vi "Start VI Helpeks.vi"() -> ()   [LabVIEW 2014]
doc: "::: VI Helpeks :::\nCopyright (c) 2000-2026 Konstantin Shifershteyn. All rights reserved."
uses:
  <vilib>/Utility/sysdir.llb/System Directory Type.ctl
  <vilib>/Platform/browser.llb/Open URL in Default Browser (string).vi
panel:
  out "LV Version":string="."
  out "Progress":i32(slide)=-1 caption="Loading . . ." scale=-1.0..380.0
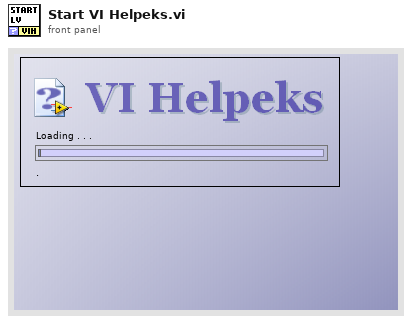
[diagram p1: front panel]
types:
  T1 = cluster{"Left Button Key Shortcut":cluster{"Control":bool, "Shift":bool, "Key":string}, "Center Button Key Shortcut":cluster{"Control":bool, "Shift":bool, "Key":string}, "Right Button Key Shortcut":cluster{"Control":bool, "Shift":bool, "Key":string}}
  T2 = enum32{"Invalid", "Standard", "Closed", "Hidden", "Minimized", "Maximized"}
  T3 = typedef "System Directory Type.ctl" = i32
  T4 = enum16{"Left Button", "Center Button", "Right Button", "Window Close"}
  T5 = typedef "NI_FileType.lvlib/LVFileType.ctl" = enum32{"Invalid file", "Unknown type", "Instrument", "Control", "Polymorphic VI", "Project", "Library", "LVClass", "XControl", "XNode", "Shared library", ".NET assembly", "ActiveX interface", "CIN", "Run-time menu", "Palette menu", "Help file", "LLB", "XNode Edit Dependency", "Class Private Data Control", "Statechart", "MathScript .m file", "Ladder Diagram", "LVLibp", "XNode Build Dependency"}
  T6 = cluster{"path":path, "delimited name":string, "type":T5, "iState":u32, "iStyle":u16, "wStyle":u16, "buttons":u16, "viflags":u32, "viflags2":u32, "links":u32[]}[]
  T7 = enum32{"Bad", "Idle", "Run top level", "Running"}
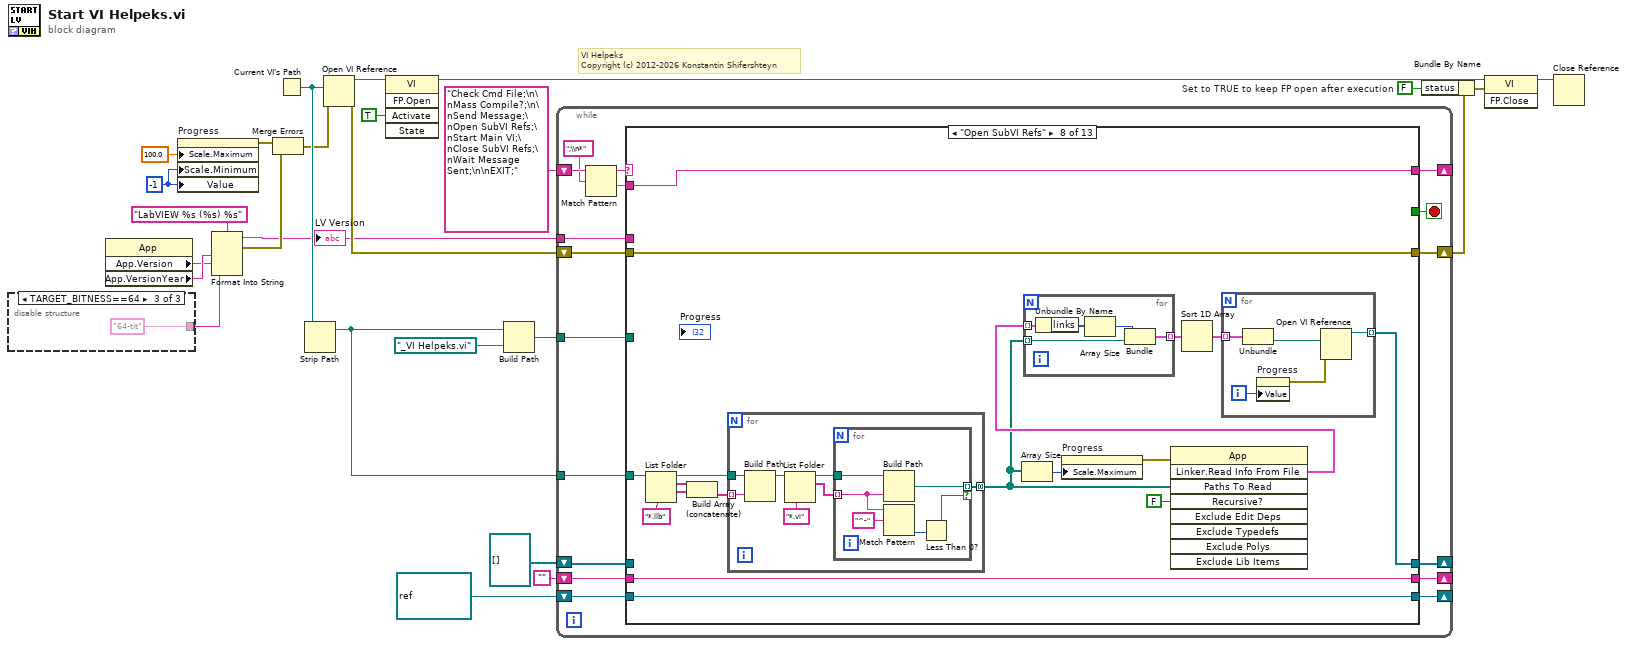
[diagram p0: block diagram]
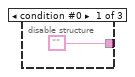
[diagram p2: hidden frame]
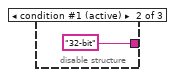
[diagram p3: hidden frame]
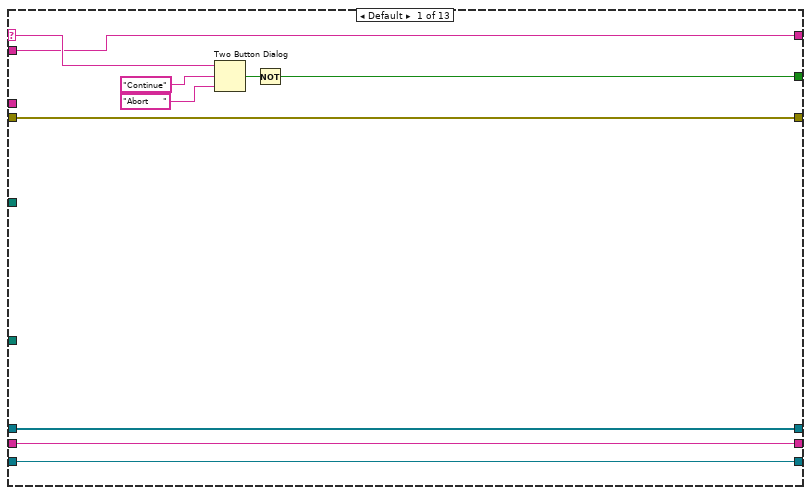
[diagram p4: hidden frame]
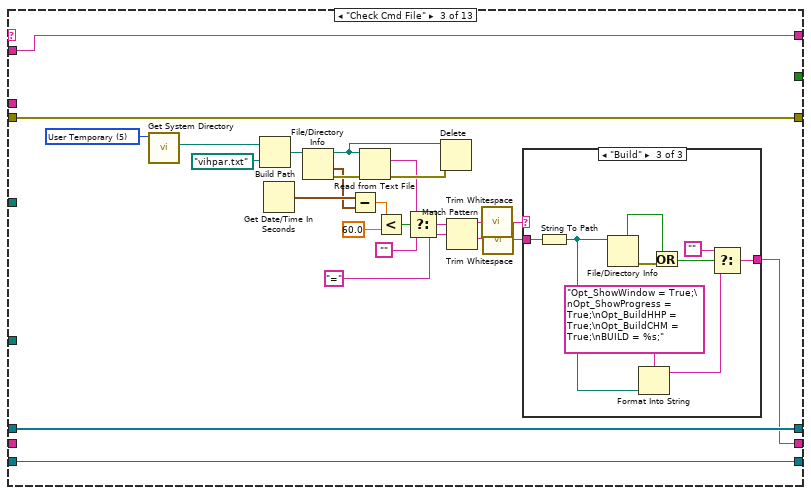
[diagram p6: hidden frame]
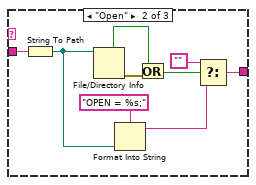
[diagram p8: hidden frame]
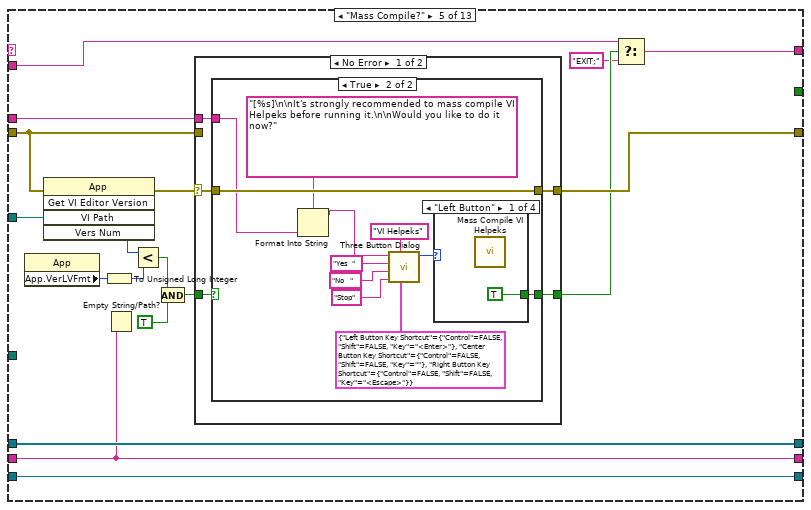
[diagram p10: hidden frame]
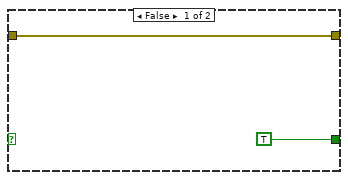
[diagram p11: hidden frame]
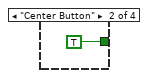
[diagram p12: hidden frame]
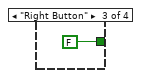
[diagram p13: hidden frame]
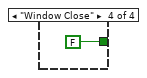
[diagram p14: hidden frame]
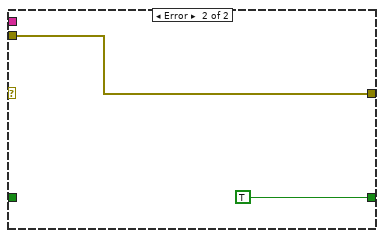
[diagram p15: hidden frame]
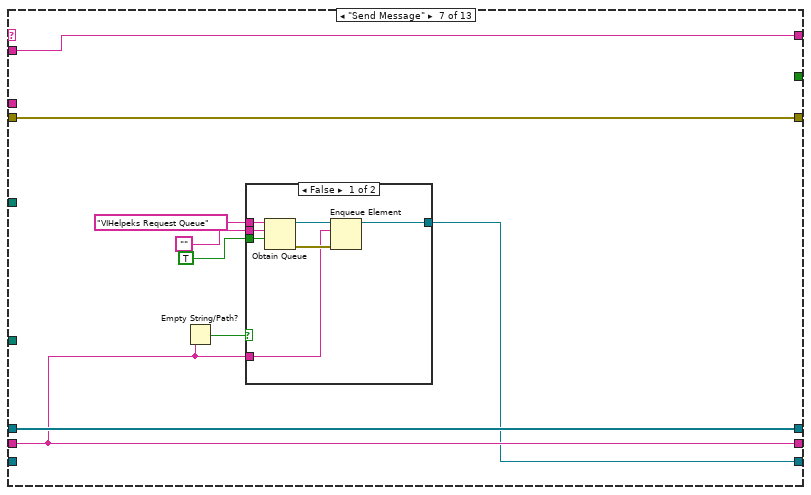
[diagram p17: hidden frame]
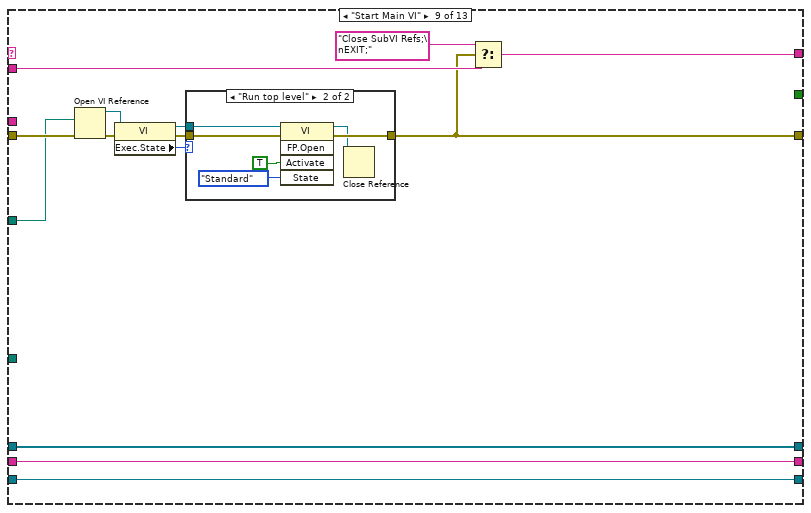
[diagram p19: hidden frame]
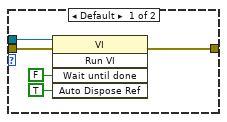
[diagram p20: hidden frame]
diagram:
  w18 = -1 ("Progress")
  w23 = FALSE  # Set to TRUE to keep FP open after execution
  # "VI Helpeks\nCopyright (c) 2012-2026 Konstantin Shifershteyn"
  n1 = disable-structure shown="TARGET_BITNESS==64" {
    disable-tunnel: ["" "32-bit" "64-tit"] -> w6
    frame condition #0 {
    }
    frame condition #1 (active) {
    }
    frame condition #2 {
    }
  }
  n2 = property class="App"() -> ("App.Version"=w9:string, "App.VersionYear"=w10:string)  [unwired: 2 in, 2 out]
  n3 = property on="Progress" class="Slide (strict)"("Scale.Maximum"=100.0 ("Scale.Range:Maximum"), "Scale.Minimum"=w18, "Value"=w18) -> (error out=w17:errorcluster)  [unwired: 2 in, 1 out]
  n4 = Format Into String(format string="LabVIEW %s (%s) %s" ("string"), w10, w9, w6) -> (resulting string=w2:string, error out=w12:errorcluster)  [unwired: 2 in]
  "LV Version" <- w2
  n5 = Merge Errors(w17, w12) -> (w13:errorcluster)
  n6 = Current VI's Path() -> (path=w26:path)
  n7 = Strip Path(path=w26) -> (stripped path=w1:path)  [unwired: 1 out]
  n8 = Open VI Reference(vi path=w26, error in (no error)=w13) -> (vi reference=w5:refnum<vi>, error out=w20:errorcluster)  [unwired: 4 in]
  n9 = invoke class="VI" method="FP.Open"(reference=w5, "Activate"=TRUE ("Activate?")) -> (reference out=w4:refnum<vi>)  [unwired: 3 in, 4 out]
  n10 = Build Path(base path=w1, name or relative path=path "_VI Helpeks.vi") -> (appended path=w21:path)
  n11 = while {
    tunnel: w21 -> [w44]
    tunnel: w1 -> [w43]
    shift-right: [w46] -> w25
    shift-left: w20 -> [w45]
    shift-right: [w42] -> _
    shift-left: refnum<vi>[] [] -> [w41]
    shift-right: [w38] -> _
    shift-left: "Check Cmd File;\n\nMass Compile?;\n\nSend Message;\nOpen SubVI Refs;\nStart Main VI;\nClose SubVI Refs;\nWait Message Sent;\n\nEXIT;" -> [w40]
    shift-right: [w33] -> _
    shift-left: "" -> [w34]
    shift-right: [w32] -> _
    shift-left: refnum<queue> refnum ("queue out") -> [w31]
    tunnel: w2 -> [w30]
    stop <- w35 stop-if-true
    n12 = Match Pattern(string=w40, regular expression=";\\n*") -> (before substring=w39:string, after substring=w37:string)  [unwired: 1 in, 2 out]
    n13 = case shown="\"Open SubVI Refs\"" w39 {
      selector: w39 -> [w55 _ _ _ _ _ _ _ _ _ _ _ _]
      tunnel: [w56 w60 w86 w108 w121 w155 w163 w184 w217 w242 w249 w276 w278] -> w46
      tunnel: w45 -> [w56 w60 w86 w108 w122 w155 w163 w184 w227 w242 w249 w276 w278]
      tunnel: w44 -> [_ _ _ _ w116 _ _ _ w226 _ _ _ _]
      tunnel: w43 -> [_ _ _ _ _ _ _ w177 _ _ _ _ _]
      tunnel: [w54 w59 w84 w107 w127 w154 w165 w185 w220 refnum<vi>[] [] w251 w275 w283] -> w42
      tunnel: w41 -> [w54 w59 w84 w107 w127 w154 w165 _ w220 w244 w251 w275 w283]
      tunnel: [w53 w61 w85 w109 w118 w156 w164 w181 w218 w241 w250 w277 w281] -> w38
      tunnel: w37 -> [w53 w61 w85 w109 w119 w156 w164 w181 w219 w241 w250 w277 w281]
      tunnel: [w49 _ _ _ _ _ _ _ _ _ _ _ TRUE] -> w35
      tunnel: w34 -> [w51 w58 _ w106 w113 w153 w162 w180 w215 w240 w247 w274 w280]
      tunnel: [w51 w58 w65 w106 w113 w153 w162 w180 w215 w240 w247 w274 w280] -> w33
      tunnel: [w47 w57 w64 w105 w111 w152 w157 w179 w214 w239 w246 w273 w279] -> w32
      tunnel: w31 -> [w47 w57 w64 w105 w111 w152 _ w179 w214 w239 w246 w273 w279]
      tunnel: w30 -> [_ _ _ _ w110 _ _ _ _ _ _ _ _]
      frame Default {
        n14 = Two Button Dialog(message=w55, 1:"Abort     ", 2:"Continue") -> (T button?=w52:bool)
        n15 = Not(x=w52) -> (.not. x?=w49:bool)
      }
      frame "" {
      }
      frame "Check Cmd File" {
        w62 = T3 5 items=["User Home"=0, "User Desktop"=1, "User Documents"=2, "User Application Data"=3, "User Preferences"=4, "User Temporary"=5, "Public Documents"=6, "Public Application Data"=7, "Public Preferences"=8, "Public Cache"=13, "System Core Libraries"=9, "System Installed Libraries"=10, "Application Files"=11, "Boot Volume Root"=12] ("system directory type")
        n16 = call <vilib>:"Get System Directory.vi"("system directory type"=w62) -> ("system directory"=w63:path)  [unwired: 10 in]
        n17 = Build Path(base path=w63, name or relative path=path "vihpar.txt") -> (appended path=w82:path)
        n18 = Get Date/Time In Seconds() -> (seconds since 1Jan1904=w78:timestamp)
        n19 = File/Directory Info(path=w82) -> (path out=w80:path, last mod=w77:timestamp, error out=w81:errorcluster)  [unwired: 1 in, 4 out]
        n20 = Subtract(x=w78, y=w77) -> (x-y=w76:dbl)
        n21 = Read from Text File(file (use dialog)=w80, error in=w81) -> (text=w73:string, error out=w79:errorcluster)  [unwired: 2 in, 2 out]
        n22 = Less?(x=w76, y=60.0) -> (x < y?=w74:bool)
        n23 = Select(t=w73, s=w74, f="") -> (s? t:f=w71:string)
        n24 = Delete(path (use dialog)=w80, error in=w79) -> ()  [unwired: 3 in, 3 out]
        n25 = Match Pattern(string=w71, regular expression="=") -> (before substring=w69:string, after substring=w67:string)  [unwired: 1 in, 2 out]
        n26 = call <vilib>:"Trim Whitespace.vi"("string"=w69) -> ("trimmed string"=w68:string)  [unwired: 1 in]
        n27 = call <vilib>:"Trim Whitespace.vi"("string"=w67) -> ("trimmed string"=w66:string)  [unwired: 1 in]
        n28 = case shown="\"Build\"" w68 {
          tunnel: w66 -> [_ w95 w104]
          tunnel: [_ w91 w100] -> w65
          frame Default {
          }
          frame "Open" {
            n29 = String To Path(string=w95) -> (path=w90:path)
            n30 = File/Directory Info(path=w90) -> (directory=w87:bool, error out=w89:errorcluster)  [unwired: 1 in, 5 out]
            n31 = Format Into String(format string="OPEN = %s;", w90) -> (resulting string=w93:string)  [unwired: 2 in, 1 out]
            n32 = Or(x=w87, y=w89) -> (x .or. y?=w88:bool)
            n33 = Select(t="", s=w88, f=w93) -> (s? t:f=w91:string)
          }
          frame "Build" {
            n34 = String To Path(string=w104) -> (path=w99:path)
            n35 = File/Directory Info(path=w99) -> (directory=w96:bool, error out=w98:errorcluster)  [unwired: 1 in, 5 out]
            n36 = Format Into String(format string="Opt_ShowWindow = True;\nOpt_ShowProgress = True;\nOpt_BuildHHP = True;\nOpt_BuildCHM = True;\nBUILD = %s;", w99) -> (resulting string=w102:string)  [unwired: 2 in, 1 out]
            n37 = Or(x=w96, y=w98) -> (x .or. y?=w97:bool)
            n38 = Select(t="", s=w97, f=w102) -> (s? t:f=w100:string)
          }
        }
      }
      frame "--------------------- 1" {
      }
      frame "Mass Compile?" {
        n39 = property class="App"() -> ("App.VerLVFmt"=w125:i32)  [unwired: 2 in, 2 out]
        n40 = invoke class="App" method="Get VI Editor Version"(error in=w122, "VI Path"=w116) -> (error out=w123:errorcluster, "Vers Num"=w124:u32)  [unwired: 3 in, 3 out]
        n41 = To Unsigned Long Integer(number=w125) -> (unsigned 32bit integer=w126:u32)
        n42 = Empty String/Path?(string/path=w113) -> ()  [unwired: 1 out]
        n43 = Less?(x=w124, y=w126) -> (x < y?=w115:bool)
        n44 = And(x=w115, y=TRUE) -> (x .and. y?=w114:bool)
        n45 = case shown="No Error" w123 {
          selector: w123 -> [w130 _]
          tunnel: w114 -> [w132 _]
          tunnel: [w131 w151] -> w121
          tunnel: w122 -> [_ w151]
          tunnel: [w129 TRUE] -> w120
          tunnel: w110 -> [w128 _]
          frame No Error {
            n46 = case shown="True" w132 {
              tunnel: [w134 w145] -> w131
              tunnel: w130 -> [w134 w145]
              tunnel: [TRUE w139] -> w129
              tunnel: w128 -> [_ w135]
              frame False {
              }
              frame True {
                n47 = Format Into String(format string="[%s]\n\nIt's strongly recommended to mass compile VI Helpeks before running it.\n\nWould you like to do it now?", w135) -> (resulting string=w137:string)  [unwired: 2 in, 1 out]
                n48 = call <vilib>:"Three Button Dialog.vi"("Keyboard Shortcuts (Left is <Enter>)"=T1 {"Left Button Key Shortcut"={"Control"=FALSE, "Shift"=FALSE, "Key"="<Enter>"}, "Center Button Key Shortcut"={"Control"=FALSE, "Shift"=FALSE, "Key"=""}, "Right Button Key Shortcut"={"Control"=FALSE, "Shift"=FALSE, "Key"="<Escape>"}}, "Window Title (\"\")"="VI Helpeks" ("Window Title (\"\")"), "Right Button Text (\"Cancel\")"="Stop" ("Right Button Text (\"Cancel\")"), "Center Button Text (\"No\")"="No   " ("F button name (\"Cancel\")"), "Left Button Text (\"Yes\")"="Yes  " ("T button name (\"OK\")"), "message"=w137) -> ("Which Button?"=w144:T4)  [unwired: 5 in]
                n49 = case shown="\"Left Button\"" w144 {
                  tunnel: [TRUE TRUE FALSE FALSE] -> w139
                  frame "Left Button" {
                    n50 = call "Mass Compile VI Helpeks.vi"() -> ()  [unwired: 1 in]
                  }
                  frame "Center Button" {
                  }
                  frame "Right Button" {
                  }
                  frame "Window Close" {
                  }
                }
              }
            }
          }
          frame Error {
          }
        }
        n51 = Select(t=w119, s=w120, f="EXIT;") -> (s? t:f=w118:string)
      }
      frame "--------------------- 2" {
      }
      frame "Send Message" {
        n52 = Empty String/Path?(string/path=w162) -> (empty?=w158:bool)
        n53 = case shown="False" w158 {
          tunnel: "VIHelpeks Request Queue" -> [w172 _]
          tunnel: "" -> [w171 _]
          tunnel: TRUE -> [w170 _]
          tunnel: w162 -> [w167 _]
          tunnel: [w166 _] -> w157
          frame False {
            n54 = Obtain Queue(name (unnamed)=w172, element data type=w171, create if not found? (T)=w170) -> (queue out=w169:refnum<queue>, error out=w168:errorcluster)  [unwired: 2 in, 1 out]
            n55 = Enqueue Element(queue=w169, element=w167, error in (no error)=w168) -> (queue out=w166:refnum<queue>)  [unwired: 1 in, 2 out]
          }
          frame True {
          }
        }
      }
      frame "Open SubVI Refs" {
        n56 = List Folder(path=w177, pattern="*.llb") -> (path out=w176:path, filenames=w175:string[], folder names=w174:string[])  [unwired: 2 in, 1 out]
        n57 = Build Array (concatenate)(w175, w174) -> (w173:string[])
        n58 = for {
          tunnel: [w194] -> w182 mode=concatenating
          tunnel: w176 -> [w193]
          tunnel: w173 -> [w191] mode=indexing
          n59 = Build Path(base path=w193, name or relative path=w191) -> (appended path=w192:path)
          n60 = List Folder(path=w192, pattern="*.vi") -> (path out=w197:path, filenames=w195:string[])  [unwired: 2 in, 2 out]
          n61 = for {
            tunnel: w197 -> [w203]
            tunnel: w195 -> [w201] mode=indexing
            tunnel: [w202] -> w194 mode=indexing if=w198
            n62 = Build Path(base path=w203, name or relative path=w201) -> (appended path=w202:path)
            n63 = Match Pattern(string=w201, regular expression="^-") -> (offset past match=w199:i32)  [unwired: 1 in, 3 out]
            n64 = Less Than 0?(x=w199) -> (x < 0?=w198:bool)
          }
        }
        n65 = Array Size(array=w182) -> (size(s)=w190:i32)
        n66 = property on="Progress" class="Slide (strict)"("Scale.Maximum"=w190) -> (error out=w187:errorcluster)  [unwired: 2 in, 1 out]
        n67 = invoke class="App" method="Linker.Read Info From File"(error in=w187, "Paths To Read"=w182, "Recursive?"=FALSE) -> ("Linker.Read Info From File"=w183:T6)  [unwired: 6 in, 8 out]
        n68 = for {
          tunnel: w183 -> [w213] mode=indexing
          tunnel: w182 -> [w211] mode=indexing
          tunnel: [w209] -> w188 mode=indexing
          n69 = Unbundle By Name(w213) -> ("links"=w212:u32[])
          n70 = Array Size(array=w212) -> (size(s)=w210:i32)
          n71 = Bundle(w210, "appended path"=w211) -> (w209:cluster{i32, "appended path":path})  [unwired: 1 in]
        }
        n72 = Sort 1D Array(array=w188) -> (sorted array=w186:cluster{i32, "appended path":path}[])
        n73 = for {
          tunnel: w186 -> [w208] mode=indexing
          tunnel: [w204] -> w185 mode=indexing
          i -> [w206]
          n74 = Unbundle(w208) -> ("appended path"=w207:path)  [unwired: 1 out]
          n75 = property on="Progress" class="Slide (strict)"("Value"=w206) -> (error out=w205:errorcluster)  [unwired: 2 in, 1 out]
          n76 = Open VI Reference(vi path=w207, error in (no error)=w205) -> (vi reference=w204:refnum<vi>)  [unwired: 4 in, 1 out]
        }
      }
      frame "Start Main VI" {
        n77 = Open VI Reference(vi path=w226, error in (no error)=w227) -> (vi reference=w224:refnum<vi>, error out=w225:errorcluster)  [unwired: 4 in]
        n78 = property class="VI"(reference=w224, error in=w225) -> (reference out=w221:refnum<vi>, error out=w222:errorcluster, "Exec.State"=w223:T7)
        n79 = case shown="\"Run top level\"" w223 {
          tunnel: [w228 w238] -> w217
          tunnel: w222 -> [w230 w234]
          tunnel: w221 -> [w229 w235]
          frame Default {
            n80 = invoke class="VI" method="Run VI"(reference=w229, error in=w230, "Wait until done"=FALSE ("Wait Until Done"), "Auto Dispose Ref"=TRUE ("Auto Dispose Reference")) -> (error out=w228:errorcluster)  [unwired: 1 in, 4 out]
          }
          frame "Run top level" {
            n81 = invoke class="VI" method="FP.Open"(reference=w235, error in=w234, "Activate"=TRUE ("Activate?"), "State"=T2."Standard") -> (reference out=w233:refnum<vi>, error out=w238:errorcluster)  [unwired: 1 in, 3 out]
            n82 = Close Reference(reference=w233) -> ()  [unwired: 1 in, 1 out]
          }
        }
        n83 = Select(t="Close SubVI Refs;\nEXIT;", s=w217, f=w219) -> (s? t:f=w218:string)
      }
      frame "Close SubVI Refs" {
        n84 = Close Reference(reference=w244) -> ()  [unwired: 1 in, 1 out]
      }
      frame "Wait Message Sent" {
        n85 = Tick Count (ms)() -> (millisecond timer value=w248:u32)
        n86 = while {
          tunnel: w248 -> [w263]
          tunnel: w247 -> [w257]
          tunnel: [w255] -> _
          tunnel: w246 -> [w254]
          tunnel: [w252] -> w245
          i -> [w255]
          stop <- w260 stop-if-true
          n87 = Tick Count (ms)() -> (millisecond timer value=w253:u32)
          n88 = Subtract(x=w253, y=w263) -> (x-y=w262:u32)
          n89 = Greater?(x=w262, y=u32 5000) -> (0:w259:bool)
          n90 = Empty String/Path?(string/path=w257) -> (empty?=w258:bool)
          n91 = Or(x=w259, y=w258) -> (x .or. y?=w256:bool)
          n92 = case shown="False" w256 {
            selector: w256 -> [_ w272]
            tunnel: [w264 w272] -> w260
            tunnel: w257 -> [_ _]
            tunnel: w254 -> [w269 w271]
            tunnel: [w265 w271] -> w252
            frame False {
              n93 = Get Queue Status(queue=w269) -> (queue out=w265:refnum<queue>, error out=w267:errorcluster, # elements in queue=w268:i32)  [unwired: 2 in, 5 out]
              n94 = Equal To 0?(x=w268) -> (x = 0?=w266:bool)
              n95 = Or(x=w267, y=w266) -> (x .or. y?=w264:bool)
              n96 = case shown="False" w264 {
                frame False {
                  n97 = Wait (ms)(milliseconds to wait=u32 50) -> ()  [unwired: 1 out]
                }
                frame True {
                }
              }
            }
            frame True {
            }
          }
        }
        n98 = Release Queue(queue=w245) -> ()  [unwired: 2 in, 3 out]
      }
      frame "--------------------- 3" {
      }
      frame "EXIT" {
        n99 = case shown="Error" w278 {
          selector: w278 -> [_ w285]
          frame No Error {
          }
          frame Error {
            n100 = Unbundle By Name(w285) -> ("code"=w284:i32)
            n101 = case shown="1003" w284 {
              selector: w284 -> [_ w294]
              tunnel: w285 -> [w286 _]
              frame Default {
                n102 = call <vilib>:"Simple Error Handler.vi"("error in (no error)"=w286) -> ()  [unwired: 4 in, 5 out]
              }
              frame 1003 {
                n103 = Format Into String(format string="Start VI Helpeks failed with error %d.\n\nThe error may occur because evaluation period has expired\nor license file is missed or broken.\n\nClick the Activate button to check the license status or activate\nVI Helpeks now. Alternatively, you can do it later with the\n\"Help>>Activate Addons\" menu.\n\nClick the Purchase button to buy a license to use VI Helpeks.\n", w294) -> (resulting string=w292:string)  [unwired: 2 in, 1 out]
                n104 = call <vilib>:"Three Button Dialog.vi"("Keyboard Shortcuts (Left is <Enter>)"=T1 {"Left Button Key Shortcut"={"Control"=FALSE, "Shift"=FALSE, "Key"="<Enter>"}, "Center Button Key Shortcut"={"Control"=FALSE, "Shift"=FALSE, "Key"=""}, "Right Button Key Shortcut"={"Control"=FALSE, "Shift"=FALSE, "Key"="<Escape>"}}, "Window Title (\"\")"="VI Helpeks" ("Window Title (\"\")"), "Right Button Text (\"Cancel\")"="Cancel    ", "Center Button Text (\"No\")"="Purchase ", "Left Button Text (\"Yes\")"="Activate  ", "message"=w292) -> ("Which Button?"=w288:T4)  [unwired: 5 in]
                n105 = case shown="\"Left Button\"" w288 {
                  frame "Left Button" {
                    n106 = invoke class="App" method="UI.Invoke Menu Item"("ItemTag"="APP_SC_ACTIVATE_ADDONS") -> ()  [unwired: 3 in, 4 out]
                  }
                  frame "Center Button" {
                    n107 = call-poly <vilib>:"Open URL in Default Browser.vi"("URL"="http://kshif.com/vihelpeks/purchase.html") -> ()  [unwired: 5 in, 2 out]
                  }
                  frame Default {
                  }
                }
              }
            }
          }
        }
      }
    }
  }
  n108 = Bundle By Name(cluster=w25, "status"=w23) -> (w24:errorcluster)
  n109 = invoke class="VI" method="FP.Close"(reference=w4, error in=w24) -> (reference out=w22:refnum<vi>)  [unwired: 1 in, 2 out]
  n110 = Close Reference(reference=w22) -> ()  [unwired: 1 in, 1 out]
